vi "Test Generate Mock Class Inherits from Mock.vi"(8 "error in (no error)":errorcluster, 11 "Test Case In":refnum<class "_Mock Class Generator Test.lvclass">) -> (0 "error out":errorcluster, 3 "Test Case Out":refnum<class "_Mock Class Generator Test.lvclass">)   [LabVIEW 2020, in "_Mock Class Generator Test.lvclass"]
uses:
  _Mock Class Generator Test.lvclass
  _Mock Class Generator Test.lvclass/_Mock Class Generator Test.ctl
  source/Scripting/Mock Class Generator/Mock Class Generator.lvclass
  d61b9b24-4b0f-44ef-a9bb-4996cb077d5f.vi
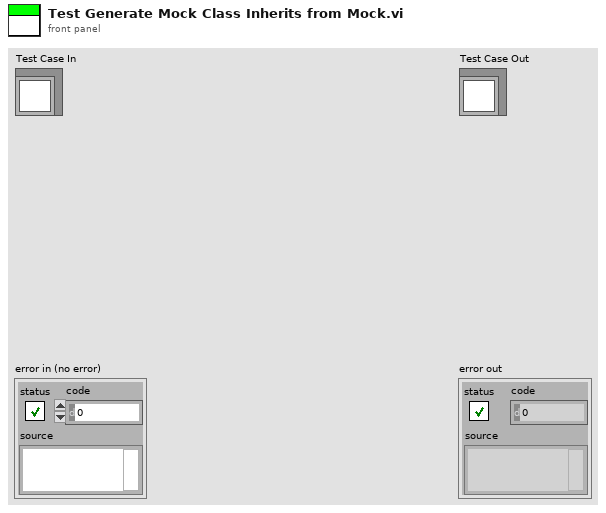
[diagram p1: front panel]
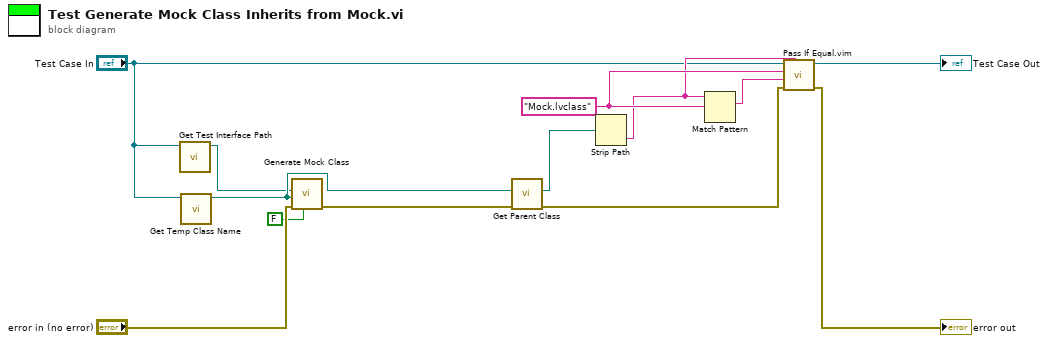
[diagram p0: block diagram]
diagram:
  w4 = "Mock.lvclass" ("regular expression")
  n1 = call "Get Test Interface Path.vi"("Mock Class Generator Test in"="Test Case In") -> ("Test Class Path"=w7:path)  [unwired: 10 in]
  n2 = call "Get Temp Class Name.vi"("Mock Class Generator Test in"="Test Case In") -> ("Test Class Path"=w10:path)  [unwired: 10 in]
  n3 = call "Generate Mock Class.vi"("Add to lvproj?"=FALSE, "error in (no error)"="error in (no error)", "Destination Class Path"=w10, "Source Class Path"=w7) -> ("error out"=w9:errorcluster)  [unwired: 6 in, 1 out]
  n4 = call "Get Parent Class.vi"("error in (no error)"=w9, "Test Class Path"=w10) -> ("error out"=w1:errorcluster, "Path"=w8:path)  [unwired: 8 in]
  n5 = Strip Path(path=w8) -> (name=w3:string)  [unwired: 1 out]
  n6 = Match Pattern(string=w3, regular expression=w4) -> (match substring=w5:string)  [unwired: 1 in, 3 out]
  n7 = call "Pass If Equal.vim"("Description"=w3, "error in (no error)"=w1, "Actual"=w5, "Expected"=w4, "LUnit Test Case In"="Test Case In") -> ("error out"=→"error out":errorcluster, "LUnit Test Case Out"=→"Test Case Out":refnum<class "_Mock Class Generator Test.lvclass">)  [unwired: 5 in]
